vi "Update.vi"(8 "error in (no error)":errorcluster, 10 "Audio Data In":dbl[][](array[numeric]), 11 "Crusher in":refnum<class "Crusher.lvclass">) -> (0 "error out":errorcluster, 2 "Audio Data Out":dbl[][](array[numeric]), 3 "Crusher out":refnum<class "Crusher.lvclass">)   [LabVIEW 2019, in "Crusher.lvlib" / "Crusher.lvclass"]
doc: "Applies bit crusher type effects. The audio signal is reduced in both sampling frequency and bit depth, producing a harsh, digital sound.\n\n<b>Value1:</b> Sampling frequency reduction factor\n<b>Value2:</b> Bit depth (1-16)"
uses:
  Crusher.lvclass
  <vilib>/Analysis/2dsp.llb/Decimate (single shot, DBL).vi
  <vilib>/gmath/NI_Gmath.lvlib
  <vilib>/Analysis/NI_AALPro.lvlib
  Plugin Interfaces/Effect Interface/Effect Interface.lvlibp/Effect Interface Class/Effect Interface.lvclass
  C:/github/dataflowg/dataflow-dj/src/Plugin Interfaces/Effect Interface/Effect Interface.lvlibp/Effect Interface Class/Effect Interface.lvclass
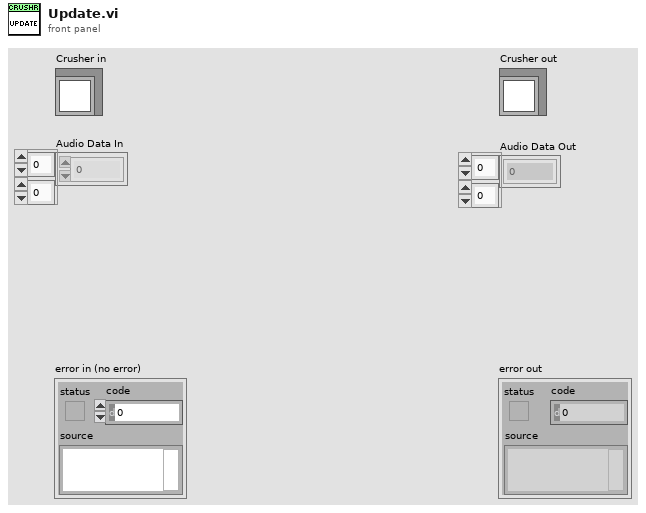
[diagram p1: front panel]
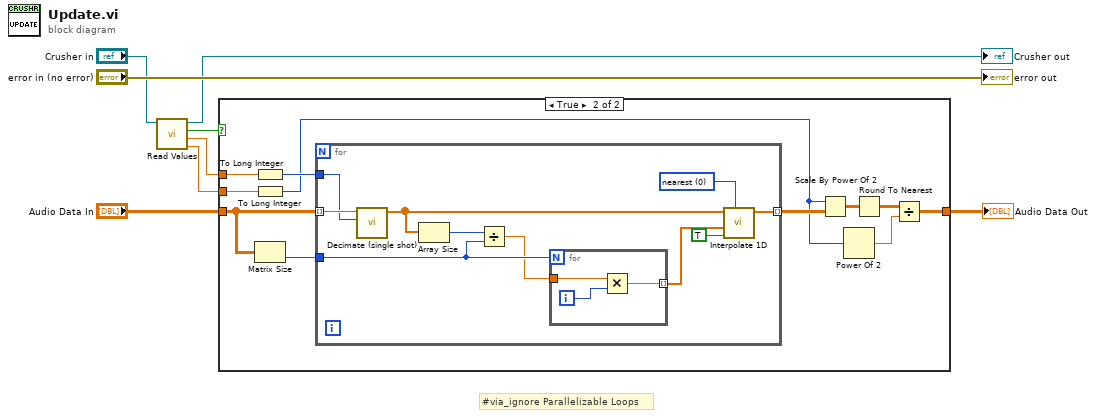
[diagram p0: block diagram]
diagram:
  # "#via_ignore Parallelizable Loops"
  n1 = call "Read Values.vi"("Effect Interface in"="Crusher in") -> ("Value2"=w1:dbl, "Value1"=w2:dbl, "Enable"=w3:bool, "Effect Interface out"=→"Crusher out":refnum<class "Crusher.lvclass">)  [unwired: 7 in]
  n2 = case shown="True" w3 {
    tunnel: w2 -> [_ w13]
    tunnel: w1 -> [_ w12]
    tunnel: "Audio Data In" -> [w9 w11]
    tunnel: [w9 w10] -> w6
    frame False {
    }
    frame True {
      n3 = To Long Integer(number=w13) -> (32bit integer=w15:i32)
      n4 = To Long Integer(number=w12) -> (32bit integer=w14:i32)
      n5 = Matrix Size(0:w11) -> (2:w20:i32)  [unwired: 1 out]
      n6 = for {
        tunnel: w11 -> [w30] mode=indexing
        tunnel: w15 -> [w29]
        tunnel: w20 -> [w27]
        tunnel: [w21] -> w19 mode=indexing
        w22 = 0 items=["nearest", "linear", "spline", "cubic Hermite", "Lagrange"] ("method")
        n7 = call-poly <vilib>:"Decimate (single shot).vi"("decimating factor"=w29, "X"=w30) -> ("Decimated Array"=w23:dbl[])  [unwired: 8 in, 1 out]
        n8 = Array Size(array=w23) -> (size(s)=w28:i32)
        n9 = Divide(x=w28, y=w27) -> (x/y=w26:dbl)
        n10 = for {
          N: w27 -> [_]
          tunnel: w26 -> [w33]
          tunnel: [w31] -> w25 mode=indexing
          i -> [w32]
          n11 = Multiply(x=w33, y=w32) -> (x*y=w31:dbl)
        }
        n12 = call <vilib>:"Interpolate 1D.vi"("method"=w22, "X is monotonic"=TRUE, "xi"=w25, "Y"=w23) -> ("yi"=w21:dbl[])  [unwired: 5 in, 2 out]
      }
      n13 = Scale By Power Of 2(n=w14, x=w19) -> (x*2^n=w18:dbl[][])
      n14 = Power Of 2(x=w14) -> (2^x=w16:dbl)
      n15 = Round To Nearest(number=w18) -> (nearest integer value=w17:dbl[][])
      n16 = Divide(x=w17, y=w16) -> (x/y=w10:dbl[][])
    }
  }
  "Audio Data Out" <- w6
  "error out" <- "error in (no error)"
